vi "QueryFirst.vi"(6 "commandTimeout in":i32=-1, 7 "CommandType":i32(ring)=-1 items=["Text"=1, "StoredProcedure"=4, "TableDirect"=512], 8 "error in (no error)":errorcluster, 9 "DynamicParameters in":refnum<class "DynamicParameters.lvclass">, 10 "sql":string, 11 "PGJDPMapper in":refnum<class "Mapper.lvclass">) -> (0 "error out":errorcluster, 2 "Value":variant, 3 "PGJDPMapper out":refnum<class "Mapper.lvclass">)   [LabVIEW 2020, in "ORM_pgsql_jdp.lvlib" / "Mapper.lvclass"]
uses:
  Mapper.lvclass
  C:/Program Files/National Instruments/LabVIEW 2020/vi.lib/Viviota/shared/ORM.lvlibp/SqlMapper/SqlMapper.lvclass
  <vilib>/Viviota/shared/ORM.lvlibp/DynamicParameters/DynamicParameters.lvclass
  dbc/DBC.lvclass
  PGJDPParameter/Parameter.lvclass
  C:/Program Files/National Instruments/LabVIEW 2020/vi.lib/Viviota/shared/ORM.lvlibp/DynamicParameters/DynamicParameters.lvclass
  <vilib>/Viviota/shared/ORM.lvlibp/SqlMapper/Read DbConnection.vi
  dbc/Read Connection.vi
  <vilib>/Viviota/shared/ORM.lvlibp/DynamicParameters/Read ParameterNames.vi
  <vilib>/Viviota/shared/ORM.lvlibp/DynamicParameters/Read ParameterValues.vi
  <vilib>/JDP Science/PostgreSQL Library/Connection/Execute Command (Result).vi
  <vilib>/Viviota/shared/ORM.lvlibp/DbConnection/DbConnection.lvclass
  <vilib>/JDP Science/PostgreSQL Library/Connection/PQ Connection.lvclass
  PGJDPResult/Result.lvclass
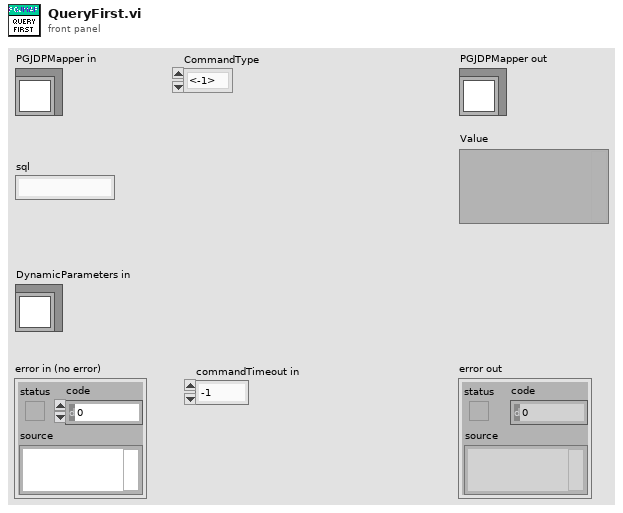
[diagram p1: front panel]
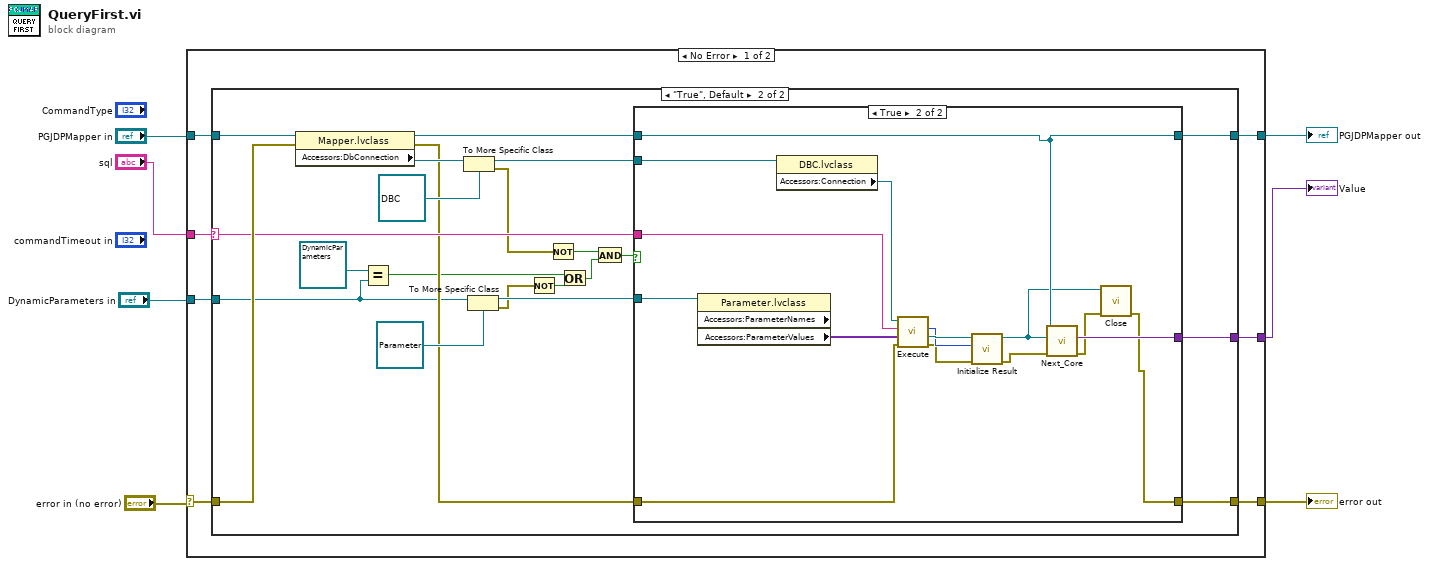
[diagram p0: block diagram]
diagram:
  n1 = case shown="No Error" "error in (no error)" {
    selector: "error in (no error)" -> [w12 w57]
    tunnel: "PGJDPMapper in" -> [w14 w56]
    tunnel: [w13 w56] -> w6
    tunnel: [w11 w57] -> w3
    tunnel: "sql" -> [w10 _]
    tunnel: "DynamicParameters in" -> [w9 _]
    tunnel: [w8 _] -> w2
    frame No Error {
      n2 = case shown="\"True\", Default" w10 {
        selector: w10 -> [_ w32]
        tunnel: w14 -> [w16 w38]
        tunnel: [w16 w26] -> w13
        tunnel: w12 -> [w15 w37]
        tunnel: [w15 w29] -> w11
        tunnel: w9 -> [_ w17]
        tunnel: [_ w28] -> w8
        frame "" {
        }
        frame "True", Default {
          n3 = property class="Mapper.lvclass"(reference=w38, error in=w37) -> (reference out=w27:refnum<class "Mapper.lvclass">, error out=w30:errorcluster, "Accessors:DbConnection"=w36:refnum<class "DbConnection.lvclass">)
          n4 = Equal?(x=refnum<class "DynamicParameters.lvclass"> refnum ("DynamicParameters"), y=w17) -> (x = y?=w23:bool)
          n5 = To More Specific Class(target class=refnum<class "DBC.lvclass"> refnum ("ORM_pgsql_jdp.lvlib:DBC.lvclass"), reference=w36) -> (specific class reference=w31:refnum<class "DBC.lvclass">, error out=w20:errorcluster)  [unwired: 1 in]
          n6 = To More Specific Class(target class=refnum<class "Parameter.lvclass"> refnum ("ORM_pgsql_jdp.lvlib:PGJDPParameter.lvclass"), reference=w17) -> (specific class reference=w33:refnum<class "Parameter.lvclass">, error out=w19:errorcluster)  [unwired: 1 in]
          n7 = Not(x=w19) -> (.not. x?=w24:bool)
          n8 = Not(x=w20) -> (.not. x?=w21:bool)
          n9 = Or(x=w23, y=w24) -> (x .or. y?=w22:bool)
          n10 = And(x=w21, y=w22) -> (x .and. y?=w18:bool)
          n11 = case shown="True" w18 {
            tunnel: w33 -> [_ w55]
            tunnel: w32 -> [_ w53]
            tunnel: w31 -> [_ w52]
            tunnel: w30 -> [w40 w50]
            tunnel: [w40 w41] -> w29
            tunnel: [_ w46] -> w28
            tunnel: w27 -> [w39 w47]
            tunnel: [w39 w47] -> w26
            frame False {
            }
            frame True {
              n12 = property class="Parameter.lvclass" props=["Accessors:ParameterNames", "Accessors:ParameterValues"](reference=w55) -> ("Accessors:ParameterValues"=w54:variant[])  [unwired: 1 in, 3 out]
              n13 = property class="DBC.lvclass"(reference=w52) -> ("Accessors:Connection"=w51:refnum<class "PQ Connection.lvclass">)  [unwired: 1 in, 2 out]
              n14 = call-poly <vilib>:"Execute.vi"("error in (no error)"=w50, "Parameter(s)"=w54, "SQL"=w53, "PQ Connection in"=w51) -> ("error out"=w45:errorcluster, "PQ Result"=w49:refnum<class "PQ Result.lvclass">, "Number of Rows"=w48:i32)  [unwired: 4 in, 1 out]
              n15 = call "Initialize Result.vi"("error in (no error)"=w45, "Count"=w48, "PQ Result"=w49) -> ("error out"=w44:errorcluster, "PGJDPResult out"=w43:refnum<class "Result.lvclass">)  [unwired: 7 in]
              n16 = call-dynamic "Next_Core.vi"("error in (no error)"=w44, "PGJDPResult in"=w43, "SqlMapper in"=w47) -> ("error out"=w42:errorcluster, "Row as Variant"=w46:variant)  [unwired: 5 in, 2 out]
              n17 = call-dynamic "Close.vi"("error in (no error)"=w42, "PGJDPResult in"=w43) -> ("error out"=w41:errorcluster)  [unwired: 9 in]
            }
          }
        }
      }
    }
    frame Error {
    }
  }
  "error out" <- w3
  "PGJDPMapper out" <- w6
  "Value" <- w2
